vi "SA set Atten Level.vi"(8 "error in (no error)":errorcluster caption="에러 입력(에러 없음)", 9 "Auto?":bool, 10 "Attenuation":dbl, 11 "Instrument Manager 입력":refnum<class "Instrument Manager.lvclass">) -> (0 "error out":errorcluster caption="에러 출력", 3 "Instrument Manager 출력":refnum<class "Instrument Manager.lvclass">)   [LabVIEW 2023, in "Instrument Manager.lvclass"]
uses:
  Instrument Manager.lvclass
  Instrument Manager.lvclass/Instrument Manager.ctl
  Module/Spectrum Analyzer/Interface_Spectrum/Interface_Spectrum.lvclass
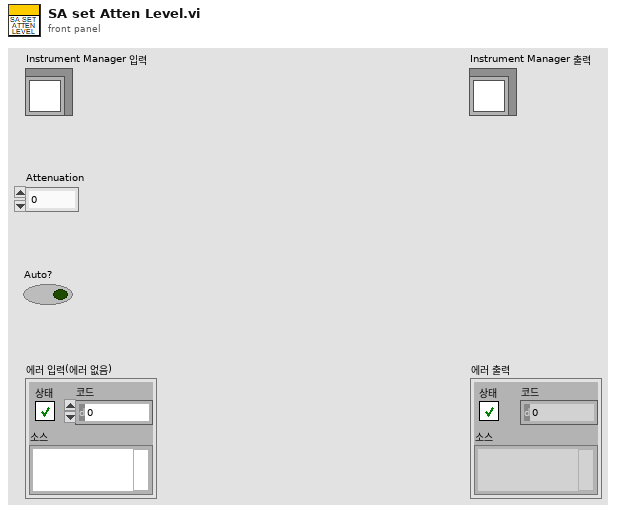
[diagram p1: front panel]
types:
  T1 = cluster{"Anritsu Call Box":refnum<class "Anritsu Call Box.lvclass">, "Spectrum Analyzer":refnum<class "Interface_Spectrum.lvclass">, "RF Switch Box":refnum<class "RF Filter Box.lvclass">, "Turn Table":refnum<class "Interface - Turn Table.lvclass">, "Mast":refnum<class "Interface - Mast.lvclass">, "3D Controller":refnum<class "Interface_3D Controller.lvclass">}
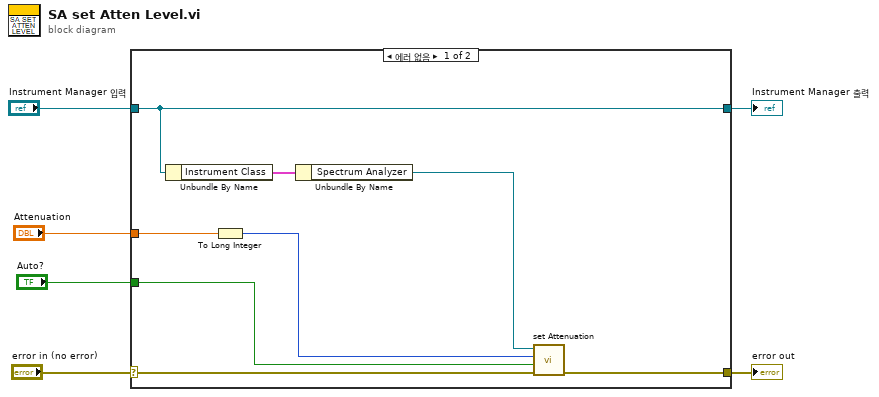
[diagram p0: block diagram]
diagram:
  n1 = case shown="에러 없음" "error in (no error)" {
    selector: "error in (no error)" -> [w11 w16]
    tunnel: [w10 w16] -> w5
    tunnel: [w14 w15] -> w3
    tunnel: "Instrument Manager 입력" -> [w14 w15]
    tunnel: "Attenuation" -> [w8 _]
    tunnel: "Auto?" -> [w9 _]
    frame No Error {
      n2 = Unbundle By Name(w14) -> ("Instrument Class"=w13:T1)
      n3 = To Long Integer(number=w8) -> (32bit integer=w7:i32)
      n4 = Unbundle By Name(w13) -> ("Spectrum Analyzer"=w12:refnum<class "Interface_Spectrum.lvclass">)
      n5 = call-dynamic "set Attenuation.vi"("error in (no error)"=w11, "Auto?"=w9, "Attenuation"=w7, "Interface_Spectrum in"=w12) -> ("error out"=w10:errorcluster)  [unwired: 6 in, 1 out]
    }
    frame Error {
    }
  }
  "error out" <- w5
  "Instrument Manager 출력" <- w3
